vi "Main.vi"() -> ()   [LabVIEW 2012]
uses:
  vi.lib/Front Panel Layout/NI_SE_Front Panel Layout.lvlib
panel:
  in  "c":bool
  in  "b":bool
  in  "a":bool
  in  "Power":bool
  out "Sensor Data":dbl[](graph)
  in  "Config Keyword":string="small1"
  in  "cancel":bool
  in  "ok":bool
  # "The following values can be used for Config Keyword:\nsmall1\nsmall2\nlarge1"
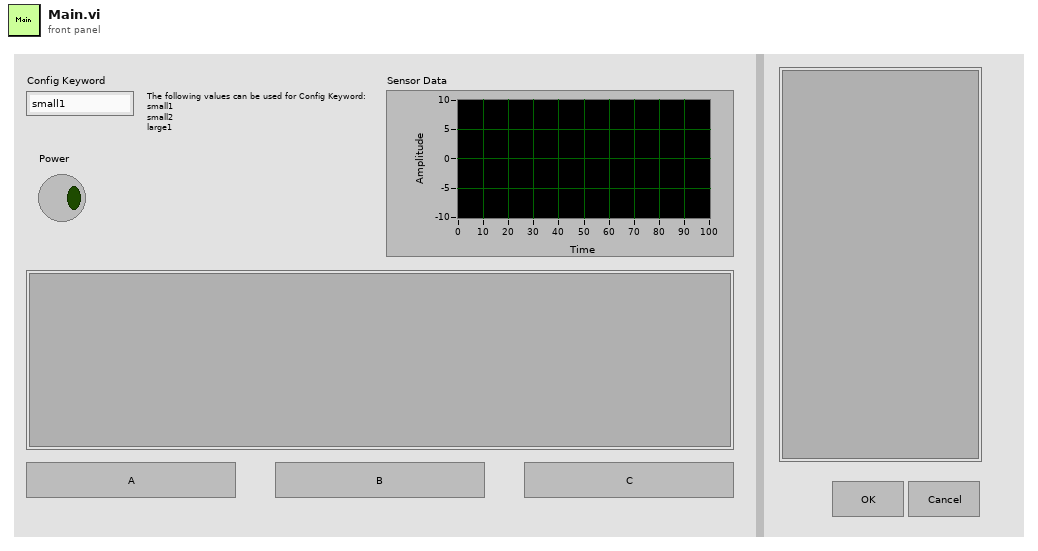
[diagram p1: front panel]
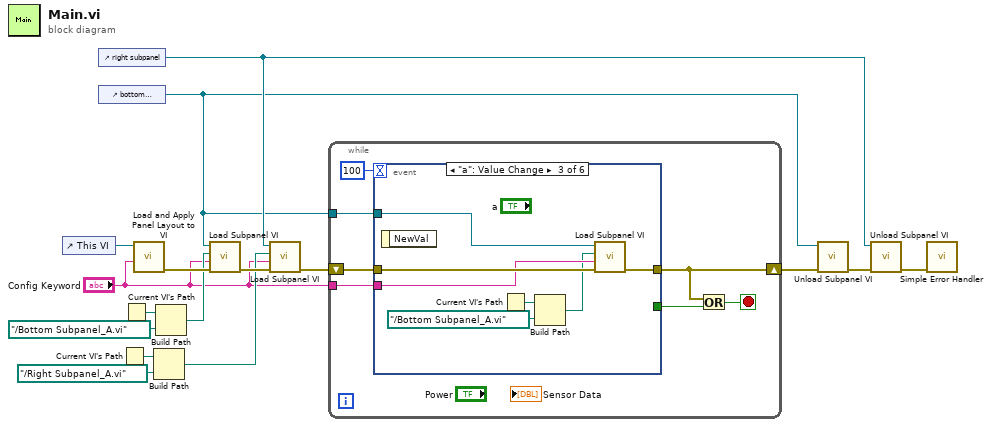
[diagram p0: block diagram]
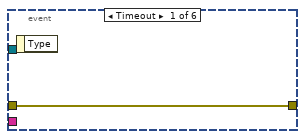
[diagram p2: hidden frame]
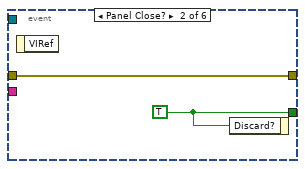
[diagram p3: hidden frame]
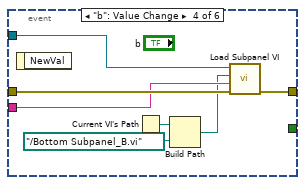
[diagram p4: hidden frame]
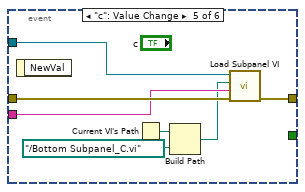
[diagram p5: hidden frame]
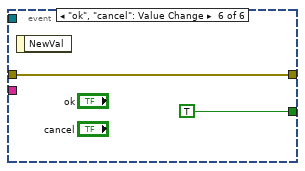
[diagram p6: hidden frame]
diagram:
  n1 = control-ref of="This VI"() -> (w16:refnum<vi>)
  n2 = control-ref of="right subpanel"() -> (w4:refnum<vi>)
  n3 = control-ref of="bottom subpanel"() -> (w3:refnum<vi>)
  n4 = Current VI's Path() -> (path=w7:path)
  n5 = Current VI's Path() -> (path=w15:path)
  n6 = call "Load and Apply Panel Layout to VI.vi"("keyword to match (\"\")"="Config Keyword", "VI refnum"=w16) -> ("error out"=w13:errorcluster)  [unwired: 8 in, 1 out]
  n7 = Build Path(base path=w7, name or relative path=path "../Right Subpanel_A.vi" ("path")) -> (appended path=w6:path)
  n8 = Build Path(base path=w15, name or relative path=path "../Bottom Subpanel_A.vi" ("path")) -> (appended path=w2:path)
  n9 = call "Load Subpanel VI.vi"("error in"=w13, "layout keyword"="Config Keyword", "subpanel VI path"=w2, "subpanel refnum"=w3) -> ("error out"=w9:errorcluster)  [unwired: 7 in]
  n10 = call "Load Subpanel VI.vi"("error in"=w9, "layout keyword"="Config Keyword", "subpanel VI path"=w6, "subpanel refnum"=w4) -> ("error out"=w8:errorcluster)  [unwired: 7 in]
  n11 = while {
    shift-right: [w17] -> w12
    shift-left: w8 -> [w23]
    tunnel: w3 -> [w19]
    tunnel: "Config Keyword" -> [w18]
    stop <- w21 stop-if-true
    n12 = event shown="[2] \"a\": Value Change" {
      selector: _ -> [_ _ _ _ _ _]
      dyn-events: _ -> [_ _ _ _ _ _]
      timeout: 100 -> [_ _ _ _ _ _]
      tunnel: w23 -> [w24 w26 w33 w40 w47 w49]
      tunnel: [w24 w26 w32 w39 w46 w49] -> w17
      tunnel: [_ w25 _ _ _ TRUE] -> w20
      tunnel: w19 -> [_ _ w30 w37 w44 _]
      tunnel: w18 -> [_ _ w31 w38 w45 _]
      event Timeout {
        n13 = event-data() -> ()  [unwired: 1 in, 1 out]
      }
      event Panel Close? {
        w25 = TRUE
        n14 = event-data() -> ()  [unwired: 1 in, 1 out]
        n15 = event-data("Discard?"=w25) -> ()  [unwired: 1 in, 1 out]
      }
      event "a": Value Change {
        n16 = event-data() -> ()  [unwired: 1 in, 1 out]
        n17 = Current VI's Path() -> (path=w29:path)
        n18 = Build Path(base path=w29, name or relative path=path "../Bottom Subpanel_A.vi" ("path")) -> (appended path=w28:path)
        n19 = call "Load Subpanel VI.vi"("error in"=w33, "layout keyword"=w31, "subpanel VI path"=w28, "subpanel refnum"=w30) -> ("error out"=w32:errorcluster)  [unwired: 7 in]
      }
      event "b": Value Change {
        n20 = event-data() -> ()  [unwired: 1 in, 1 out]
        n21 = Current VI's Path() -> (path=w36:path)
        n22 = Build Path(base path=w36, name or relative path=path "../Bottom Subpanel_B.vi" ("path")) -> (appended path=w35:path)
        n23 = call "Load Subpanel VI.vi"("error in"=w40, "layout keyword"=w38, "subpanel VI path"=w35, "subpanel refnum"=w37) -> ("error out"=w39:errorcluster)  [unwired: 7 in]
      }
      event "c": Value Change {
        n24 = event-data() -> ()  [unwired: 1 in, 1 out]
        n25 = Current VI's Path() -> (path=w43:path)
        n26 = Build Path(base path=w43, name or relative path=path "../Bottom Subpanel_C.vi" ("path")) -> (appended path=w42:path)
        n27 = call "Load Subpanel VI.vi"("error in"=w47, "layout keyword"=w45, "subpanel VI path"=w42, "subpanel refnum"=w44) -> ("error out"=w46:errorcluster)  [unwired: 7 in]
      }
      event "ok", "cancel": Value Change {
        n28 = event-data() -> ()  [unwired: 1 in, 1 out]
      }
    }
    n29 = Or(x=w17, y=w20) -> (x .or. y?=w21:bool)
  }
  n30 = call "Unload Subpanel VI.vi"("error in"=w12, "subpanel refnum"=w3) -> ("error out"=w11:errorcluster)  [unwired: 9 in]
  n31 = call "Unload Subpanel VI.vi"("error in"=w11, "subpanel refnum"=w4) -> ("error out"=w10:errorcluster)  [unwired: 9 in]
  n32 = call <vilib>:"Simple Error Handler.vi"("error in (no error)"=w10) -> ()  [unwired: 4 in, 5 out]
